vi "interface_labview.vi"() -> ()   [LabVIEW 2019]
uses:
  <vilib>/Instr/_visa.llb/VISA Configure Serial Port (Instr).vi
panel:
  out "Buzzer actif":bool
  out "Alerte":bool
  out "Système Actif":bool
  in  "Stop":bool
  in  "Boolean 2":bool
  in  "Boolean":bool
  out "Température":dbl(graph)
  out "Thermometer":dbl(slide) scale=0.0..100.0
  out "Température(°C)":dbl
  # "Panneau de Configuration"
  # "Etat du systéme"
  # "Etat du Température"
  # "Port Série"
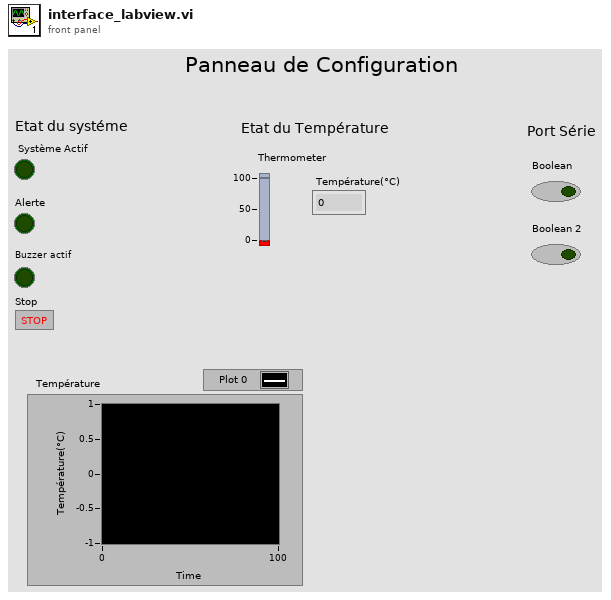
[diagram p1: front panel]
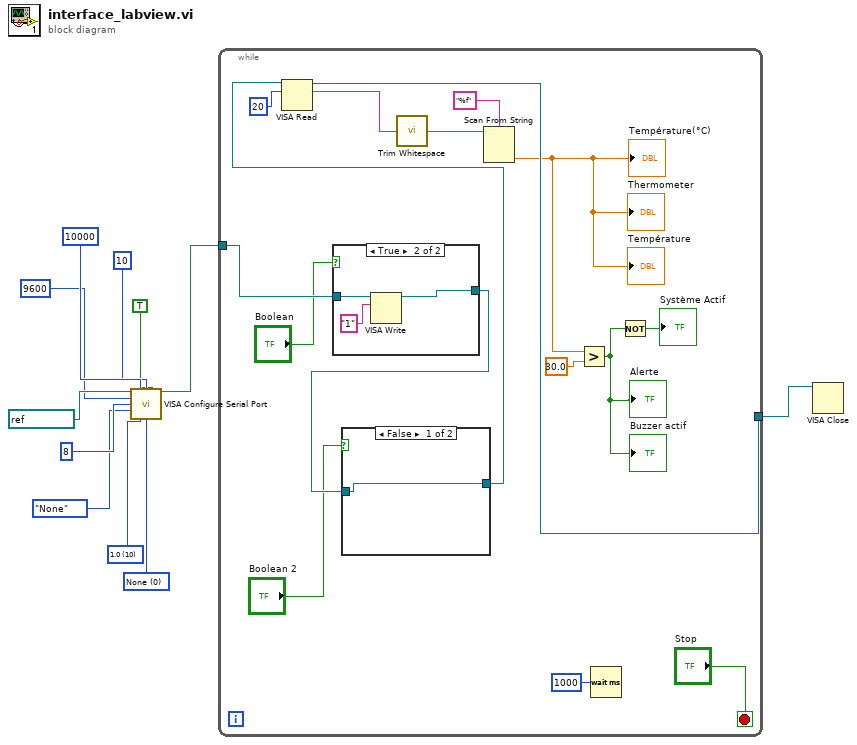
[diagram p0: block diagram]
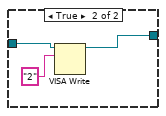
[diagram p2: hidden frame]
diagram:
  w3 = u16 0 items=["None", "XON/XOFF", "RTS/CTS", "XON/XOFF & RTS/CTS", "DTR/DSR", "XON/XOFF & DTR/DSR"] ("flow control (0:none)")
  w4 = u16 10 items=["1.0"=10, "1.5"=15, "2.0"=20] ("stop bits (10: 1 bit)")
  n1 = call-poly "VISA Configure Serial Port"("VISA resource name"=refnum<visa-resource-name> "CNCB0", "timeout (10sec)"=u32 10000, "termination char\n(0xA = '\\n' = LF)"=u8 10 ("termination char\n(0xA = '\\n' = LF)"), "Enable Termination\nChar (T)"=TRUE ("Enable Termination\nChar (T)"), "baud rate (9600)"=u32 9600, "data bits (8)"=u16 8, "parity (0:none)"=enum16{"None", "Odd", "Even", "Mark", "Space"}."None", "stop bits (10: 1 bit)"=w4, "flow control (0:none)"=w3) -> ("VISA resource name out"=w2:refnum<visa-resource-name>)  [unwired: 5 in, 1 out]
  n2 = while {
    tunnel: w2 -> [w24]
    tunnel: [w16] -> w1
    stop <- "Stop" stop-if-true
    n3 = case shown="True" "Boolean" {
      tunnel: w24 -> [w32 w35]
      tunnel: [w32 w33] -> w23
      frame False {
      }
      frame True {
        n4 = VISA Write(VISA resource name=w35, write buffer="1") -> (VISA resource name out=w33:refnum<visa-resource-name>)  [unwired: 1 in, 2 out]
      }
    }
    n5 = case shown="False" "Boolean 2" {
      tunnel: w23 -> [w28 w31]
      tunnel: [w28 w30] -> w17
      frame False {
      }
      frame True {
        n6 = VISA Write(VISA resource name=w31, write buffer="2") -> (VISA resource name out=w30:refnum<visa-resource-name>)  [unwired: 1 in, 2 out]
      }
    }
    n7 = VISA Read(VISA resource name=w17, byte count=u32 20) -> (VISA resource name out=w16:refnum<visa-resource-name>, read buffer=w27:string)  [unwired: 1 in, 2 out]
    n8 = call <vilib>:"Trim Whitespace.vi"("string"=w27) -> ("trimmed string"=w26:string)  [unwired: 1 in]
    n9 = Scan From String(format string="%f", input string=w26) -> (output 1=w15:dbl)  [unwired: 3 in, 3 out]
    "Température(°C)" <- w15
    "Thermometer" <- w15
    "Température" <- w15
    n10 = Greater?(x=w15, y=30.0) -> (0:w13:bool)
    "Alerte" <- w13
    "Buzzer actif" <- w13
    n11 = Wait (ms)(milliseconds to wait=u32 1000) -> ()  [unwired: 1 out]
    n12 = Not(x=w13) -> (.not. x?=→"Système Actif":bool)
  }
  n13 = VISA Close(VISA resource name=w1) -> ()  [unwired: 1 in, 1 out]
